vi "Write Language Selection UTF-16 LE.vi"(8 "error in (no error)":errorcluster, 10 "Langúage Selection":T1, 11 "LanguageSelection file":path) -> (0 "error out":errorcluster, 3 "text":string)   [LabVIEW 2019, in "Language Selection.lvlib"]
doc: "Convert translation from JSON format.\n- - -\nCopyright (c) 2026, Merecs Engineering GmbH"
uses:
  Language Selection.lvlib
  TypeDefs/Cluster Language Configuration.ctl
  Cluster Settings Data.ctl
  TypeDefs/Cluster Language.ctl
  TypeDefs/Cluster PropertyTranslation.ctl
  TypeDefs/Enum Property Type.ctl
  229035d7-406c-47fd-bea0-38559dbf66ce.vi
  private/Hex-String To String.vi
  <vilib>/JDP Science/JSONtext/Variant to JSON Text.vi
  <vilib>/addons/Tools/Unicode/_subVIs/Convert ASCII to UTF-16LE (Scalar).vi
  <vilib>/JDP Science/JSONtext/LVClass Serializer/JSONtext LVClass Serializer.lvclass
  <vilib>/addons/Tools/Unicode/UI Unicode Tools.lvlib
panel:
  # "Connector Pane"
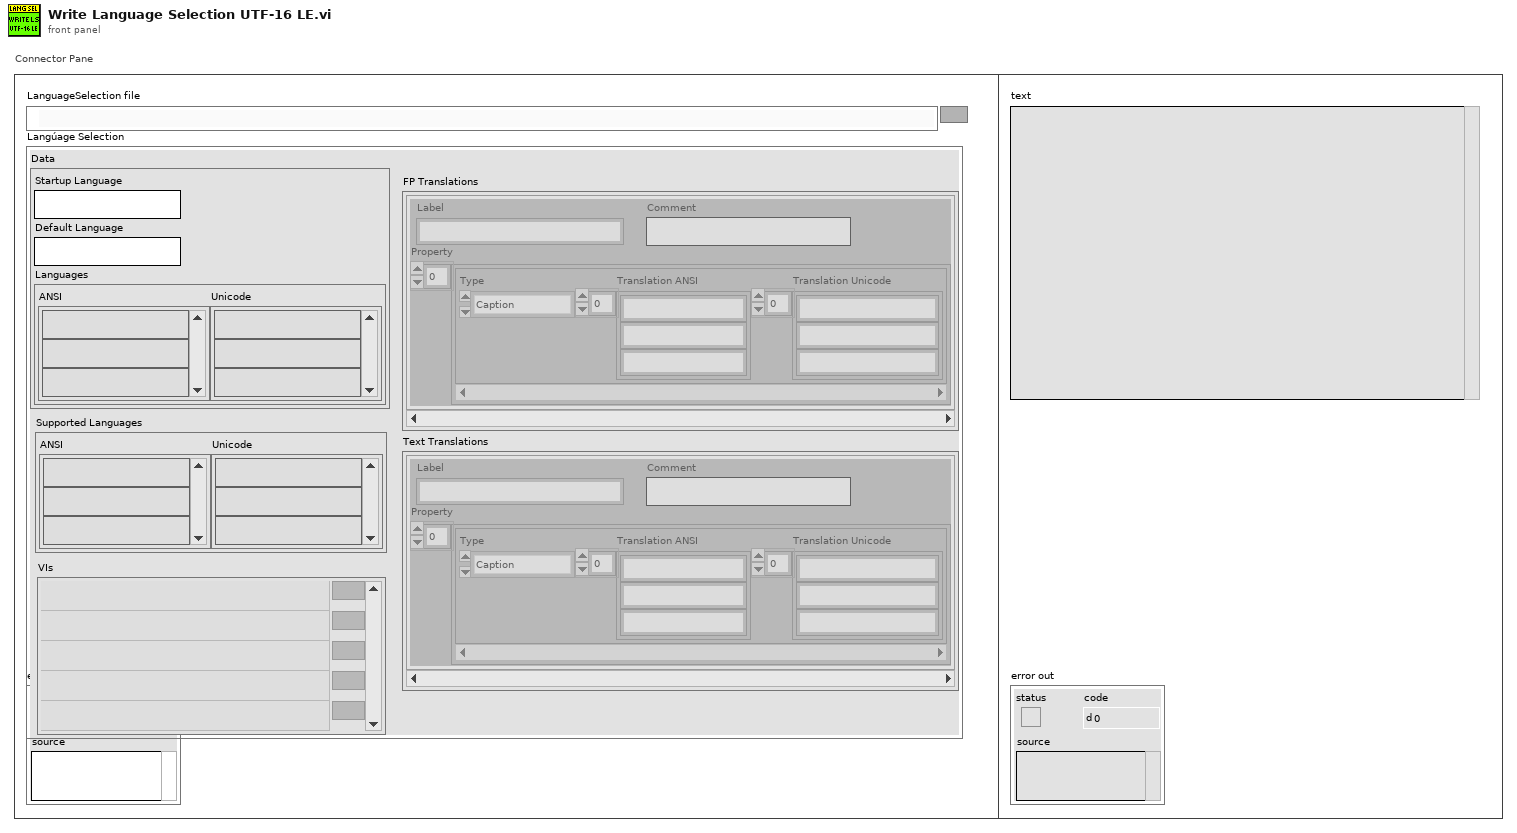
[diagram p1: front panel]
types:
  T1 = typedef "Language Selection.lvlib/Cluster Language Configuration.ctl" = cluster{"Data":T2, "Supported Languages":cluster{"ANSI":string[], "Unicode":string[]}, "VIs":path[], "FP Translations":T3[], "Text Translations":T3[]}
  T2 = typedef "Language Selection.lvlib/Cluster Settings Data.ctl" = cluster{"Startup Language":string, "Default Language":string, "Languages":cluster{"ANSI":string[], "Unicode":string[]}}
  T3 = typedef "Language Selection.lvlib/Cluster Language.ctl" = cluster{"Label":string, "Comment":string, "Property":T4[]}
  T4 = typedef "Language Selection.lvlib/Cluster PropertyTranslation.ctl" = cluster{"Type":T5, "Translation ANSI":string[], "Translation Unicode":string[]}
  T5 = typedef "Language Selection.lvlib/Enum Property Type.ctl" = enum16{"NA", "Caption", "String Value", "Boolean Text", "Ring Strings", "1D Array Elements", "2D Array Elements", "(MC)Listbox Header", "(MC)Listbox Items", "Tab Pages Names", "X & Y GraphChart", "Plot Names", "Table Headers", "Table Items", "TipStrip", "Combobox Strings", "Cursor Name", "Tree Col Headers"}
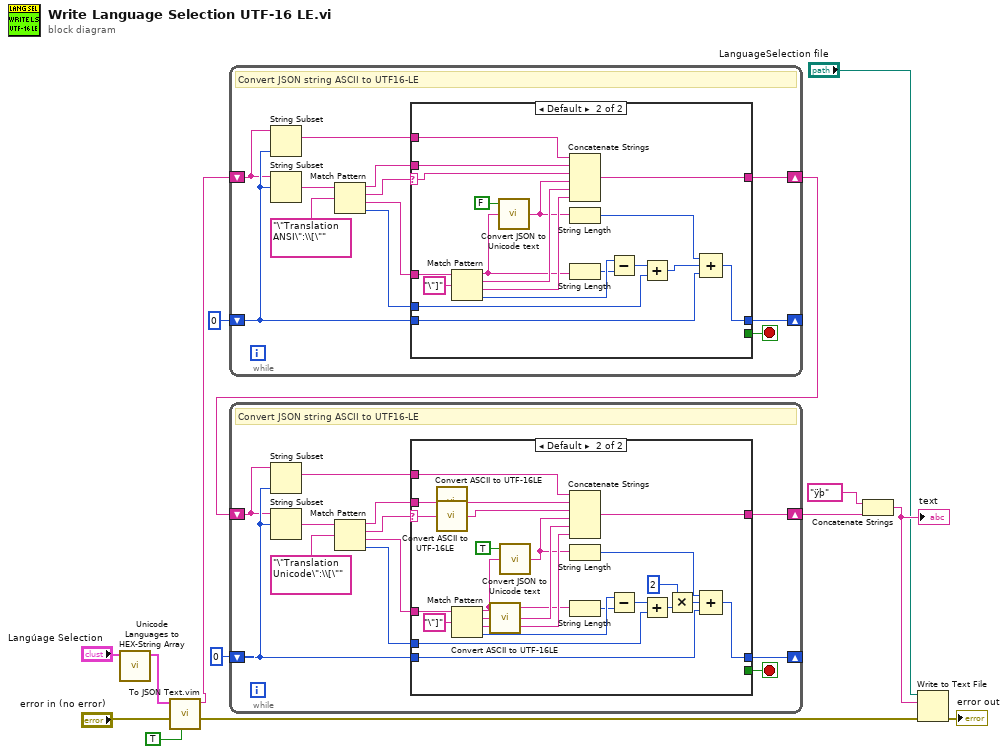
[diagram p0: block diagram]
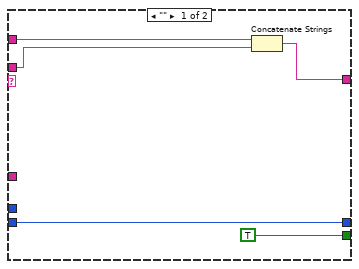
[diagram p2: hidden frame]
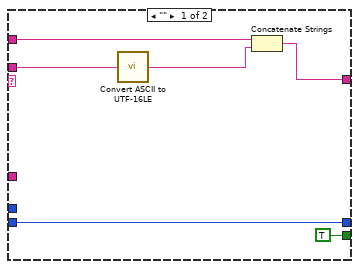
[diagram p3: hidden frame]
diagram:
  n1 = call "Unicode Languages to HEX-String Array.vi"("Config Data in"="Langúage Selection") -> ("Config Data out"=w6:T1)  [unwired: 10 in]
  n2 = call "To JSON Text.vim"("Pretty Print?"=TRUE, "error in (no error)"="error in (no error)", "Anything"=w6) -> ("error out"=w9:errorcluster, "<JSON>"=w3:string)  [unwired: 7 in]
  n3 = while {
    shift-right: [w16] -> w2
    shift-left: w3 -> [w17]
    shift-right: [w22] -> _
    shift-left: 0 -> [w18]
    stop <- w23 stop-if-true
    # "Convert JSON string ASCII to UTF16-LE"
    n4 = String Subset(string=w17, length (rest)=w18) -> (substring=w15:string)  [unwired: 1 in]
    n5 = String Subset(string=w17, offset (0)=w18) -> (substring=w19:string)  [unwired: 1 in]
    n6 = Match Pattern(string=w19, regular expression="\"Translation ANSI\":\\[\"") -> (before substring=w20:string, match substring=w24:string, after substring=w25:string, offset past match=w21:i32)  [unwired: 1 in]
    n7 = case shown="Default" w24 {
      selector: w24 -> [_ w47]
      tunnel: w25 -> [_ w50]
      tunnel: w20 -> [w27 w37]
      tunnel: [w28 w48] -> w16
      tunnel: [TRUE _] -> w23
      tunnel: [w30 w40] -> w22
      tunnel: w18 -> [w30 w36]
      tunnel: w21 -> [_ w44]
      tunnel: w15 -> [w29 w43]
      frame "" {
        n8 = Concatenate Strings(w29, w27) -> (w28:string)
      }
      frame Default {
        n9 = Match Pattern(string=w50, regular expression="\"]") -> (before substring=w35:string, match substring=w46:string, after substring=w45:string, offset past match=w42:i32)  [unwired: 1 in]
        n10 = call "Convert JSON to Unicode text.vi"("String in"=w35, "Unicode (True)"=FALSE) -> ("String out"=w34:string)  [unwired: 3 in]
        n11 = Concatenate Strings(w43, w37, w47, w34, w46, w45) -> (w48:string)
        n12 = String Length(string=w34) -> (length=w39:i32)
        n13 = String Length(string=w35) -> (length=w38:i32)
        n14 = Subtract(x=w42, y=w38) -> (x-y=w41:i32)
        n15 = Add(x=w41, y=w44) -> (x+y=w32:i32)
        n16 = Compound Arithmetic op=ADD(w39, w32, w36) -> (w40:i32)
      }
    }
  }
  n17 = while {
    shift-right: [w52] -> w1
    shift-left: w2 -> [w53]
    shift-right: [w58] -> _
    shift-left: 0 -> [w54]
    stop <- w59 stop-if-true
    # "Convert JSON string ASCII to UTF16-LE"
    n18 = String Subset(string=w53, length (rest)=w54) -> (substring=w51:string)  [unwired: 1 in]
    n19 = String Subset(string=w53, offset (0)=w54) -> (substring=w55:string)  [unwired: 1 in]
    n20 = Match Pattern(string=w55, regular expression="\"Translation Unicode\":\\[\"") -> (before substring=w56:string, match substring=w60:string, after substring=w61:string, offset past match=w57:i32)  [unwired: 1 in]
    n21 = case shown="Default" w60 {
      selector: w60 -> [_ w82]
      tunnel: w61 -> [_ w92]
      tunnel: w56 -> [w64 w75]
      tunnel: [w65 w90] -> w52
      tunnel: [TRUE _] -> w59
      tunnel: [w67 w78] -> w58
      tunnel: w54 -> [w67 w72]
      tunnel: w57 -> [_ w84]
      tunnel: w51 -> [w66 w81]
      frame "" {
        n22 = call-poly <vilib>:"Convert ASCII to UTF-16LE.vi"("ASCII"=w64) -> ("Unicode"=w63:string)  [unwired: 4 in]
        n23 = Concatenate Strings(w66, w63) -> (w65:string)
      }
      frame Default {
        n24 = call-poly <vilib>:"Convert ASCII to UTF-16LE.vi"("ASCII"=w75) -> ("Unicode"=w74:string)  [unwired: 4 in]
        n25 = call-poly <vilib>:"Convert ASCII to UTF-16LE.vi"("ASCII"=w82) -> ("Unicode"=w89:string)  [unwired: 4 in]
        n26 = Match Pattern(string=w92, regular expression="\"]") -> (before substring=w71:string, match substring=w88:string, after substring=w86:string, offset past match=w80:i32)  [unwired: 1 in]
        n27 = call-poly <vilib>:"Convert ASCII to UTF-16LE.vi"("ASCII"=w88) -> ("Unicode"=w87:string)  [unwired: 4 in]
        n28 = call "Convert JSON to Unicode text.vi"("String in"=w71, "Unicode (True)"=TRUE) -> ("String out"=w70:string)  [unwired: 3 in]
        n29 = Concatenate Strings(w81, w74, w89, w70, w87, w86) -> (w90:string)
        n30 = String Length(string=w70) -> (length=w77:i32)
        n31 = String Length(string=w71) -> (length=w76:i32)
        n32 = Subtract(x=w80, y=w76) -> (x-y=w79:i32)
        n33 = Add(x=w79, y=w84) -> (x+y=w83:i32)
        n34 = Multiply(x=2 ("y"), y=w83) -> (x*y=w73:i32)
        n35 = Compound Arithmetic op=ADD(w77, w73, w72) -> (w78:i32)
      }
    }
  }
  n36 = Concatenate Strings("ÿþ" ("string"), w1) -> (w14:string)
  "text" <- w14
  n37 = Write to Text File(file (use dialog)="LanguageSelection file", text=w14, error in=w9) -> (error out=→"error out":errorcluster)  [unwired: 1 in, 2 out]
